vi "Template Enumeration Path.vi"() -> (2 "Template Enumeration Path":path)   [LabVIEW 2020, in "LV-Protoc.lvlib"]
uses:
  LV-Protoc.lvlib
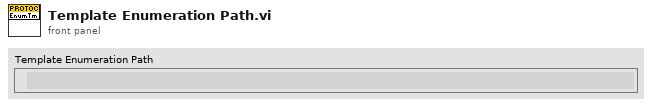
[diagram p1: front panel]
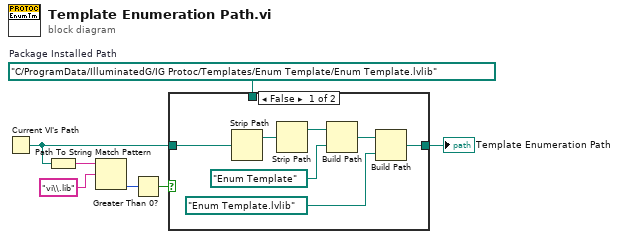
[diagram p0: block diagram]
diagram:
  w1 = path "C:/ProgramData/IlluminatedG/IG Protoc/Templates/Enum Template/Enum Template.lvlib"  # Package Installed Path
  n1 = Current VI's Path() -> (path=w5:path)
  n2 = Path To String(path=w5) -> (string=w6:string)
  n3 = Match Pattern(string=w6, regular expression="vi\\.lib") -> (offset past match=w3:i32)  [unwired: 1 in, 3 out]
  n4 = Greater Than 0?(x=w3) -> (x > 0?=w2:bool)
  n5 = case shown="False" w2 {
    tunnel: [w9 w15] -> w7
    tunnel: w5 -> [w8 _]
    tunnel: w1 -> [_ w15]
    frame False {
      n6 = Strip Path(path=w8) -> (stripped path=w14:path)  [unwired: 1 out]
      n7 = Strip Path(path=w14) -> (stripped path=w13:path)  [unwired: 1 out]
      n8 = Build Path(base path=w13, name or relative path=path "Enum Template") -> (appended path=w11:path)
      n9 = Build Path(base path=w11, name or relative path=path "Enum Template.lvlib") -> (appended path=w9:path)
    }
    frame True {
    }
  }
  "Template Enumeration Path" <- w7
